vi "Get REF StringsAndValues.vi"(8 "error in (no error)":errorcluster, 11 "Channels.REF":T1 {"Roll-Off" min=1; "TC" min=0.0001 format="%#_3p"; "Phase" format="%#_3g"; "Frequency" min=0.0001 max=200000.0 format="%#_6p"; "Channel" min=1}) -> (0 "error out":errorcluster, 2 "REF Strings and Values":cluster{string, i32}[](array[cluster]))   [LabVIEW 2019, in "Instrument.Lockin.lvlib" / "Instrument UI.Lockin.lvclass"]
uses:
  Instrument UI.Lockin.lvclass
  Instrument.DAQ/Typedefs/REF.Channel--Cluster--Array.ctl
  Instrument.DAQ/Typedefs/REF.Channel--Cluster.ctl
  Instrument.DAQ/Instrument.DAQ.lvclass
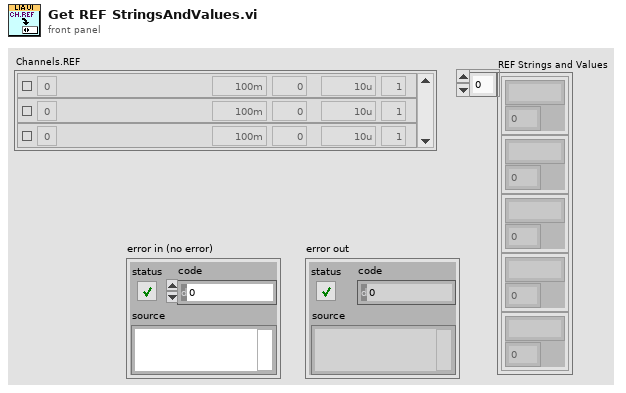
[diagram p1: front panel]
types:
  T1 = typedef "Instrument.Lockin.lvlib/Instrument.DAQ.lvclass/REF.Channel--Cluster--Array.ctl" = T2[]
  T2 = typedef "Instrument.Lockin.lvlib/Instrument.DAQ.lvclass/REF.Channel--Cluster.ctl" = cluster{"Enable?":bool, "Channel":i32, "Frequency":dbl, "Phase":dbl, "TC":dbl, "Roll-Off":i32}
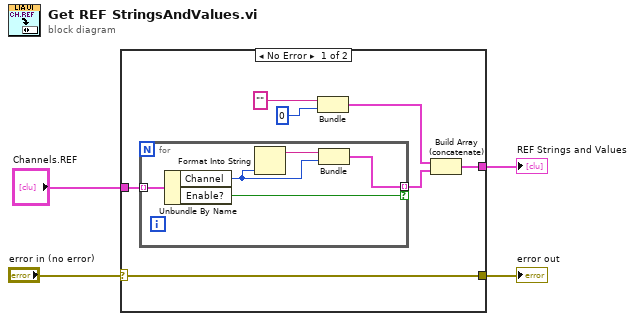
[diagram p0: block diagram]
diagram:
  n1 = case shown="No Error" "error in (no error)" {
    selector: "error in (no error)" -> [w11 w17]
    tunnel: [w7 _] -> w4
    tunnel: [w11 w17] -> w2
    tunnel: "Channels.REF" -> [w6 _]
    frame No Error {
      n2 = for {
        tunnel: w6 -> [w16] mode=indexing
        tunnel: [w12] -> w5 mode=indexing if=w15
        n3 = Unbundle By Name(w16) -> ("Channel"=w13:i32, "Enable?"=w15:bool)
        n4 = Format Into String(w13) -> (resulting string=w14:string)  [unwired: 3 in, 1 out]
        n5 = Bundle(w14, "Channel"=w13) -> (w12:cluster{string, "Channel":i32})  [unwired: 1 in]
      }
      n6 = Bundle("format string"="", "x+1"=0) -> (w8:cluster{"format string":string, "x+1":i32})  [unwired: 1 in]
      n7 = Build Array (concatenate)(w8, w5) -> (w7:cluster{"format string":string, "Channel":i32}[])
    }
    frame Error {
    }
  }
  "REF Strings and Values" <- w4
  "error out" <- w2
